vi "RemoteVI Loop Greeting.vi"(0 "context":T2, 5 "state":T1) -> (4 "greeting":string, 6 "overlay frame":string, 8 "hWnd":u64, 10 "html":string, 14 "view only?":bool, 15 "token":string)   [LabVIEW 2020, in "RemoteVI.lvlib"]
doc: "What a client accepted in this iteration of the server loop gets first: the greeting followed by the origin, tips and splitters messages as WebSocket text frames, plus what RemoteVI Accept Clients.vi needs besides: the overlay last sent, the window handle, the page, the access token and view only."
uses:
  RemoteVI.lvlib
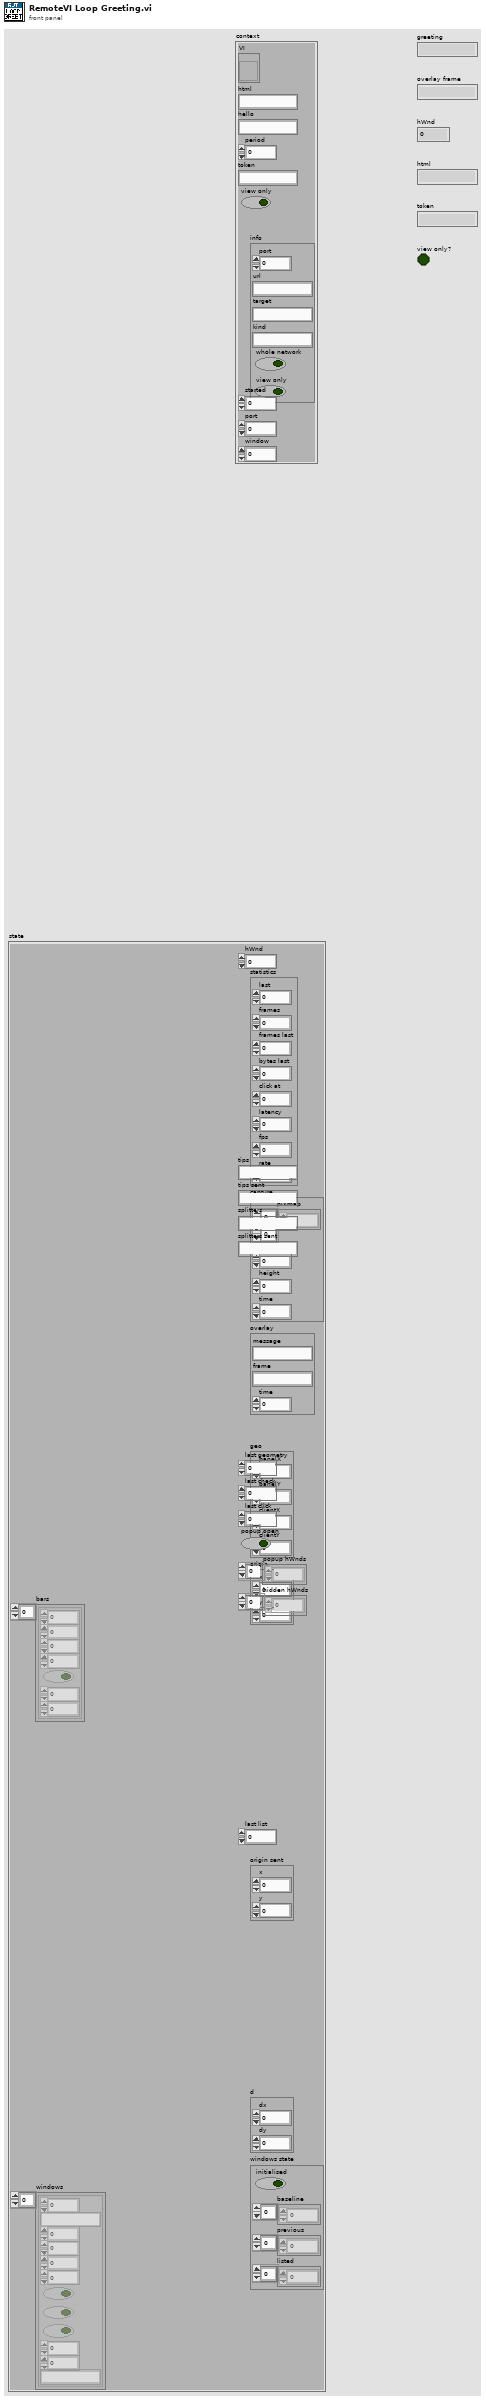
[diagram p1: front panel]
types:
  T1 = cluster{"statistics":cluster{"last":dbl, "frames":u32, "frames last":u32, "bytes last":dbl, "click at":dbl, "latency":dbl, "fps":dbl, "rate":dbl}, "capture":cluster{"pixmap":u32[][], "width":i32, "height":i32, "time":u32}, "overlay":cluster{"message":string, "frame":string, "time":u32}, "hWnd":u64, "geo":cluster{"panelX":i32, "panelY":i32, "clientX":i32, "clientY":i32}, "origin":cluster{"x":i32, "y":i32}, "tips":string, "tips sent":string, "splitters":string, "splitters sent":string, "bars":cluster{"x":i32, "y":i32, "w":i32, "h":i32, "vertical":bool, "min":i32, "max":i32}[], "origin sent":cluster{"x":i32, "y":i32}, "last geometry":u32, "last check":u32, "last click":u32, "popup open":bool, "popup hWnds":u64[], "hidden hWnds":u64[], "d":cluster{"dx":i32, "dy":i32}, "windows state":cluster{"initialised":bool, "baseline":u64[], "previous":u64[], "listed":u64[]}, "last list":u32, "windows":cluster{"id":u64, "title":string, "x":i32, "y":i32, "w":i32, "h":i32, "modal":bool, "active":bool, "closable":bool, "sx":i32, "sy":i32, "class":string}[]}
  T2 = cluster{"VI":refnum<vi>, "html":string, "hello":string, "period":dbl, "token":string, "view only":bool, "info":cluster{"port":u16, "url":string, "target":string, "kind":string, "whole network":bool, "view only":bool}, "started":dbl, "port":u16, "window":u64}
  T3 = cluster{"message":string, "frame":string, "time":u32}
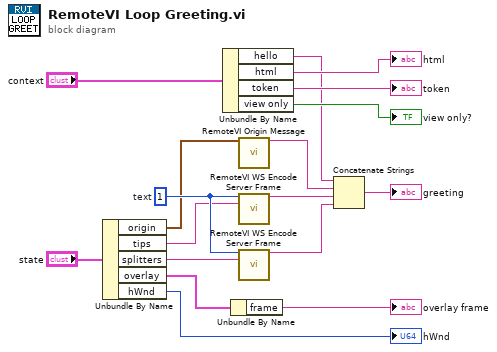
[diagram p0: block diagram]
diagram:
  w14 = u8 1  # text
  n1 = Unbundle By Name("state") -> ("origin"=w7:cluster{"x":i32, "y":i32}, "tips"=w8:string, "splitters"=w9:string, "overlay"=w10:T3, "hWnd"=→"hWnd":u64)
  n2 = Unbundle By Name("context") -> ("hello"=w2:string, "html"=→"html":string, "token"=→"token":string, "view only"=→"view only?":bool)
  n3 = Unbundle By Name(w10) -> ("frame"=→"overlay frame":string)
  n4 = call "RemoteVI Origin Message.vi"("origin"=w7) -> ("frame"=w13:string)  [unwired: 14 in]
  n5 = call "RemoteVI WS Encode Server Frame.vi"("opcode"=w14, "payload"=w8) -> ("frame"=w15:string)  [unwired: 13 in]
  n6 = call "RemoteVI WS Encode Server Frame.vi"("opcode"=w14, "payload"=w9) -> ("frame"=w16:string)  [unwired: 13 in]
  n7 = Concatenate Strings(w2, w13, w15, w16) -> (→"greeting":string)
